vi "VIH HelpGen - HTML - Find Allowed HTML Tag (Initial or Final).vi"(8 "Offset":i32, 10 "Tags (upper case)":string[](array[string]), 11 "String":string) -> (0 "Offset out":i32, 1 "After":string, 2 "Match":string, 3 "Before":string)   [LabVIEW 2014]
doc: "::: VI Helpeks :::\nCopyright (c) 2000-2026 Konstantin Shifershteyn. All rights reserved."
panel:
  # "VI Helpeks\nCopyright (c) 2012-2026 Konstantin Shifershteyn"
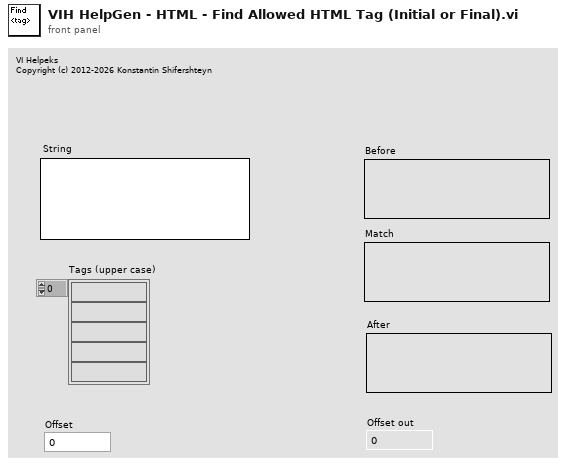
[diagram p1: front panel]
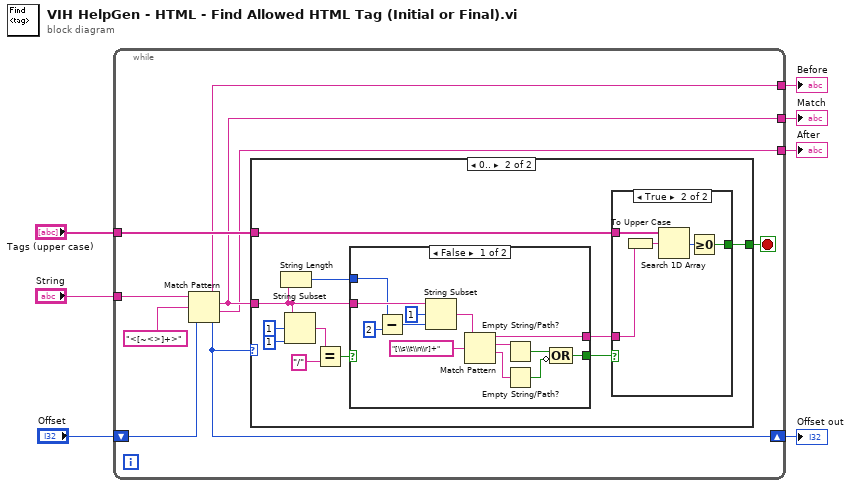
[diagram p0: block diagram]
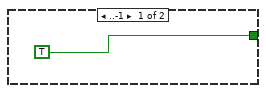
[diagram p2: hidden frame]
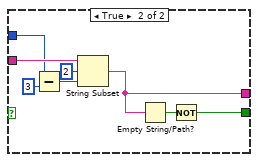
[diagram p4: hidden frame]
diagram:
  n1 = while {
    tunnel: "Tags (upper case)" -> [w14]
    tunnel: "String" -> [w15]
    shift-right: [w12] -> w1
    shift-left: "Offset" -> [w13]
    tunnel: [w10] -> w4
    tunnel: [w9] -> w3
    tunnel: [w8] -> w2
    stop <- w11 stop-if-true
    n2 = Match Pattern(string=w15, regular expression="<[~<>]+>", offset (0)=w13) -> (before substring=w10:string, match substring=w9:string, after substring=w8:string, offset past match=w12:i32)
    n3 = case shown="0.." w12 {
      tunnel: w9 -> [_ w20]
      tunnel: w14 -> [_ w23]
      tunnel: [TRUE w22] -> w11
      frame ..-1 {
      }
      frame 0.. {
        n4 = String Length(string=w20) -> (length=w19:i32)
        n5 = String Subset(string=w20, offset (0)=1, length (rest)=1 ("length (rest)")) -> (substring=w26:string)
        n6 = Equal?(x=w26, y="/" ("x")) -> (x = y?=w21:bool)
        n7 = case shown="False" w21 {
          tunnel: w20 -> [w46 w53]
          tunnel: [w43 w49] -> w24
          tunnel: w19 -> [w40 w50]
          tunnel: [w34 w47] -> w18
          frame False {
            n8 = Subtract(x=w40, y=2) -> (x-y=w41:i32)
            n9 = String Subset(string=w46, offset (0)=1, length (rest)=w41) -> (substring=w44:string)
            n10 = Match Pattern(string=w44, regular expression="[\\s\\t\\n\\r]+") -> (before substring=w43:string, match substring=w38:string, after substring=w37:string)  [unwired: 1 in, 1 out]
            n11 = Empty String/Path?(string/path=w38) -> (empty?=w36:bool)
            n12 = Empty String/Path?(string/path=w37) -> (empty?=w35:bool)
            n13 = Compound Arithmetic op=OR(w36, invert w35) -> (w34:bool)
          }
          frame True {
            n14 = Subtract(x=w50, y=3) -> (x-y=w51:i32)
            n15 = String Subset(string=w53, offset (0)=2, length (rest)=w51) -> (substring=w49:string)
            n16 = Empty String/Path?(string/path=w49) -> (empty?=w48:bool)
            n17 = Not(x=w48) -> (.not. x?=w47:bool)
          }
        }
        n18 = case shown="True" w18 {
          tunnel: w24 -> [_ w33]
          tunnel: w23 -> [_ w32]
          tunnel: [_ w30] -> w22
          frame False {
          }
          frame True {
            n19 = To Upper Case(1:w33) -> (0:w29:string)
            n20 = Search 1D Array(1D array=w32, element=w29) -> (index of element=w31:i32)  [unwired: 1 in]
            n21 = Greater Or Equal To 0?(x=w31) -> (x >= 0?=w30:bool)
          }
        }
      }
    }
  }
  "Before" <- w4
  "Match" <- w3
  "After" <- w2
  "Offset out" <- w1
